vi "Setup.vi"(11 "error in":errorcluster) -> (4 "Application Ref":refnum<vi>, 6 "VI Reference Out":refnum<vi>, 15 "error out":errorcluster)   [LabVIEW 2016, in "Drona.lvlib"]
doc: "Initiates the launcher VI as specified in Drona configuration file and return its application & VI reference."
uses:
  Drona.lvlib
  _Typedefs/SetupSourceConfig.ctl
  _Typedefs/SetupEXEConfig.ctl
  <vilib>/Utility/error.llb/Error Cluster From Error Code.vi
  Get/GetVI/GetVIByPath.vi
  Stimulus/VI/OpenVIFrontPanel.vi
  Stimulus/VI/RunVI.vi
  Get/GetVI/GetVIByName.vi
  <vilib>/ErrorRing/Error Ring.xnode
  Get/GetVI/GetVI.lvlib
  <vilib>/Utility/config.llb/NI_LVConfig.lvlib
  <vilib>/SLL Toolkit/SLL File IO/SLL File IO.lvlib
  Stimulus/VI/VI.lvlib
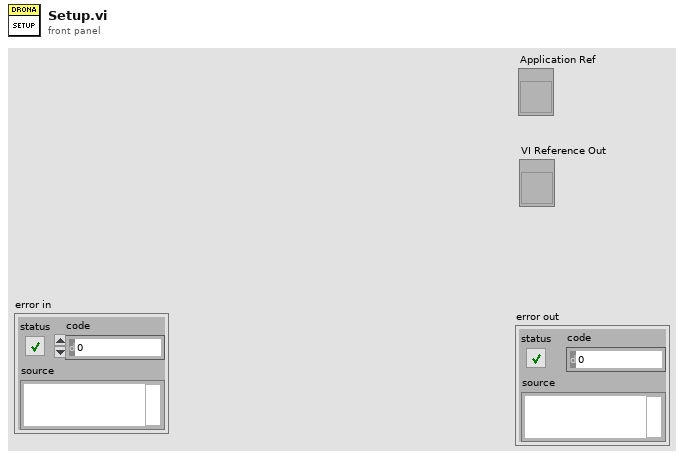
[diagram p1: front panel]
types:
  T1 = typedef "Drona.lvlib/SetupSourceConfig.ctl" = cluster{"LauncherPath":path, "Open?":bool, "Run?":bool}
  T2 = typedef "NI_LVConfig.lvlib/Config Data RefNum.ctl" = refnum<k1>
  T3 = enum32{"Bad", "Idle", "Run top level", "Running"}
  T4 = typedef "Drona.lvlib/SetupEXEConfig.ctl" = cluster{"LauncherName":string}
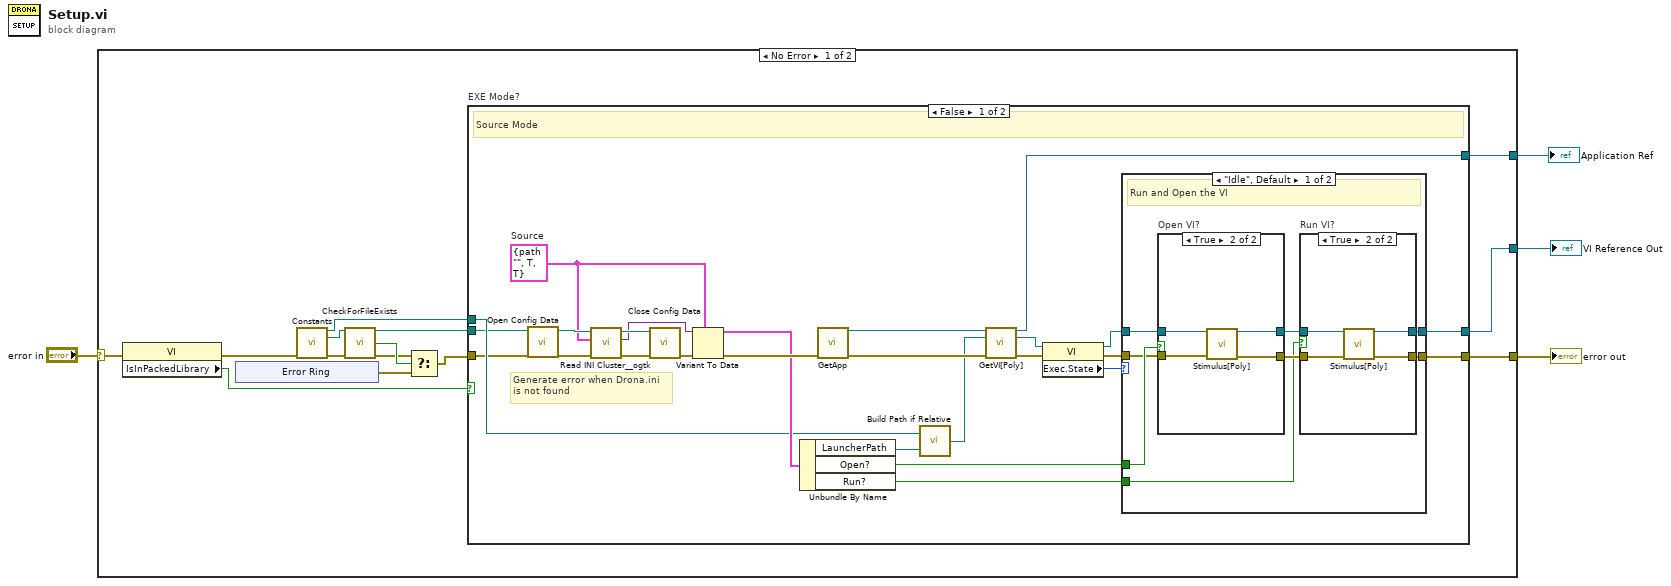
[diagram p0: block diagram]
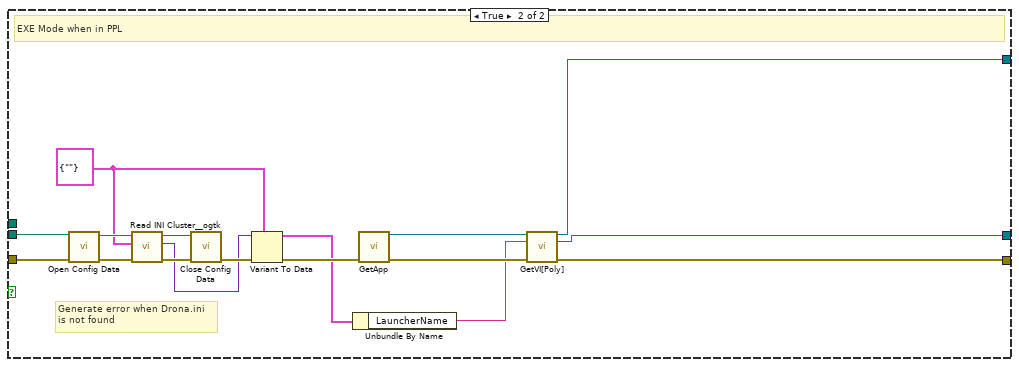
[diagram p5: hidden frame]
diagram:
  n1 = case shown="No Error" "error in" {
    selector: "error in" -> [w15 w89]
    tunnel: [w18 _] -> w3
    tunnel: [w17 _] -> w2
    tunnel: [w16 w89] -> w1
    frame No Error {
      n2 = property class="VI"(error in=w15) -> (error out=w13:errorcluster, "IsInPackedLibrary"=w14:bool)  [unwired: 1 in, 1 out]
      n3 = xnode "Error Ring"() -> ("error out"=w9:errorcluster)
      n4 = call "Constants.vi"("error in"=w13) -> ("Source path"=w5:path, "Drona ini file path"=w6:path, "error out"=w12:errorcluster)  [unwired: 12 in]
      n5 = call "CheckForFileExists.vi"("Path"=w6, "error in"=w12) -> ("Dup Path"=w11:path, "File Exists?"=w10:bool, "error out"=w8:errorcluster)  [unwired: 11 in]
      n6 = Select(t=w8, s=w10, f=w9) -> (s? t:f=w7:errorcluster)
      n7 = case "EXE Mode?" shown="False" w14 {
        tunnel: [w44 w83] -> w18
        tunnel: [w43 w82] -> w17
        tunnel: [w42 w86] -> w16
        tunnel: w7 -> [w24 w73]
        tunnel: w11 -> [w25 w72]
        tunnel: w5 -> [w26 _]
        frame False {
          w27 = T1 {"LauncherPath"=path "", "Open?"=TRUE, "Run?"=TRUE}  # Source
          # "Generate error when Drona.ini\nis not found"
          # "Source Mode"
          n8 = call <vilib>:"Open Config Data.vi"("error in (no error)"=w24, "configuration file path"=w25) -> ("error out"=w32:errorcluster, "refnum"=w31:T2)  [unwired: 7 in, 1 out]
          n9 = call <userlib>:"Read INI Cluster__ogtk.vi"("error in (no error)"=w32, "INI Fomatted Cluster Type"=w27, "refnum"=w31) -> ("error out"=w33:errorcluster, "INI Fomatted Cluster"=w28:variant, "dup refnum"=w29:T2)  [unwired: 4 in, 2 out]
          n10 = call <vilib>:"Close Config Data.vi"("error in (no error)"=w33, "refnum"=w29) -> ("error out"=w30:errorcluster)  [unwired: 8 in, 1 out]
          n11 = Variant To Data(error in=w30, type=w27, Variant=w28) -> (data=w45:T1, error out=w46:errorcluster)
          n12 = Unbundle By Name(w45) -> ("LauncherPath"=w35:path, "Open?"=w41:bool, "Run?"=w40:bool)
          n13 = call "GetApp.vi"("error in (no error)"=w46) -> ("Application Ref"=w48:refnum<vi>, "error out"=w49:errorcluster)  [unwired: 13 in]
          n14 = call <vilib>:"Build Path if Relative.vi"("Relative or Absolute Path"=w35, "Base Path"=w26) -> ("Path Out"=w34:path)
          n15 = call-poly "GetVI[Poly].vi"("Application Ref in"=w48, "VI Path"=w34, "error in (no error)"=w49) -> ("Application Ref out"=w44:refnum<vi>, "VI Reference"=w38:refnum<vi>, "error out"=w47:errorcluster)  [unwired: 10 in]
          n16 = property class="VI"(reference=w38, error in=w47) -> (reference out=w37:refnum<vi>, error out=w39:errorcluster, "Exec.State"=w36:T3)
          n17 = case shown="\"Idle\", Default" w36 {
            tunnel: [w55 w70] -> w43
            tunnel: [w54 w71] -> w42
            tunnel: w41 -> [w53 _]
            tunnel: w40 -> [w52 _]
            tunnel: w39 -> [w51 w71]
            tunnel: w37 -> [w50 w70]
            frame "Idle", Default {
              # "Run and Open the VI"
              n18 = case "Open VI?" shown="True" w53 {
                tunnel: [w64 w66] -> w57
                tunnel: [w65 w68] -> w56
                tunnel: w51 -> [w64 w67]
                tunnel: w50 -> [w65 w69]
                frame False {
                }
                frame True {
                  n19 = call-poly "Stimulus[Poly].vi"("VI Reference In"=w69, "error in"=w67) -> ("VI Reference Out"=w68:refnum<vi>, "error out"=w66:errorcluster)  [unwired: 12 in]
                }
              }
              n20 = case "Run VI?" shown="True" w52 {
                tunnel: w57 -> [w58 w62]
                tunnel: w56 -> [w59 w63]
                tunnel: [w59 w61] -> w55
                tunnel: [w58 w60] -> w54
                frame False {
                }
                frame True {
                  n21 = call-poly "Stimulus[Poly].vi"("VI Reference In"=w63, "error in"=w62) -> ("VI Reference Out"=w61:refnum<vi>, "error out"=w60:errorcluster)  [unwired: 12 in]
                }
              }
            }
            frame "Run top level" {
              # "Already Running"
            }
          }
        }
        frame True {
          w74 = T4 {"LauncherName"=""} ("EXE")
          # "Generate error when Drona.ini\nis not found"
          # "EXE Mode when in PPL"
          n22 = call <vilib>:"Open Config Data.vi"("error in (no error)"=w73, "configuration file path"=w72) -> ("error out"=w79:errorcluster, "refnum"=w78:T2)  [unwired: 7 in, 1 out]
          n23 = call <userlib>:"Read INI Cluster__ogtk.vi"("error in (no error)"=w79, "INI Fomatted Cluster Type"=w74, "refnum"=w78) -> ("error out"=w80:errorcluster, "INI Fomatted Cluster"=w75:variant, "dup refnum"=w76:T2)  [unwired: 4 in, 2 out]
          n24 = call <vilib>:"Close Config Data.vi"("error in (no error)"=w80, "refnum"=w76) -> ("error out"=w77:errorcluster)  [unwired: 8 in, 1 out]
          n25 = Variant To Data(error in=w77, type=w74, Variant=w75) -> (data=w84:T4, error out=w85:errorcluster)
          n26 = Unbundle By Name(w84) -> ("LauncherName"=w81:string)
          n27 = call "GetApp.vi"("error in (no error)"=w85) -> ("Application Ref"=w87:refnum<vi>, "error out"=w88:errorcluster)  [unwired: 13 in]
          n28 = call-poly "GetVI[Poly].vi"("Application Ref in"=w87, "VI Name"=w81, "error in (no error)"=w88) -> ("Application Ref out"=w83:refnum<vi>, "VI Reference"=w82:refnum<vi>, "error out"=w86:errorcluster)  [unwired: 10 in]
        }
      }
    }
    frame Error {
    }
  }
  "error out" <- w1
  "VI Reference Out" <- w2
  "Application Ref" <- w3
